vi "RemoteVI Server Share.vi"(0 "row":T1, 1 "port":u16=8100, 2 "whole network?":bool, 3 "view only?":bool, 8 "token":string) -> (4 "URL":string, 5 "message":string, 15 "error out":errorcluster)   [LabVIEW 2020, in "RemoteVI.lvlib"]
doc: "RemoteVI Server's Share button: shares the window of row. A panel of a RUNNING VI of this application instance (RemoteVI VI Of Window.vi) is shared as a VI target (RemoteVI Start.vi: tip strips and splitter dragging work); every other window - of another LabVIEW, a built application or any program, or the panel of a VI that is not running - as a window target (RemoteVI Start Window.vi). message is one line for the UI: the link, or why it failed (port in use, port shared already)."
uses:
  RemoteVI.lvlib
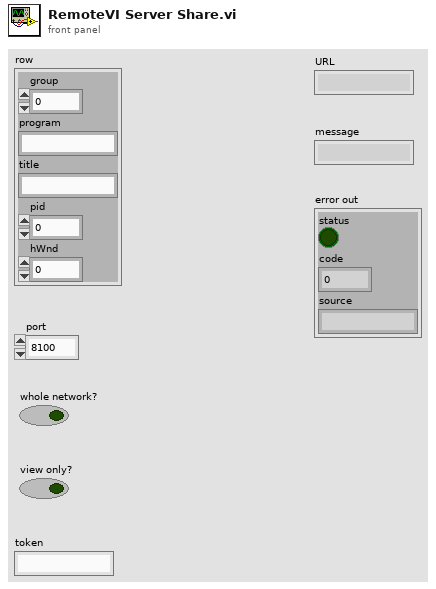
[diagram p1: front panel]
types:
  T1 = cluster{"group":i32, "program":string, "title":string, "pid":u32, "hWnd":u64}
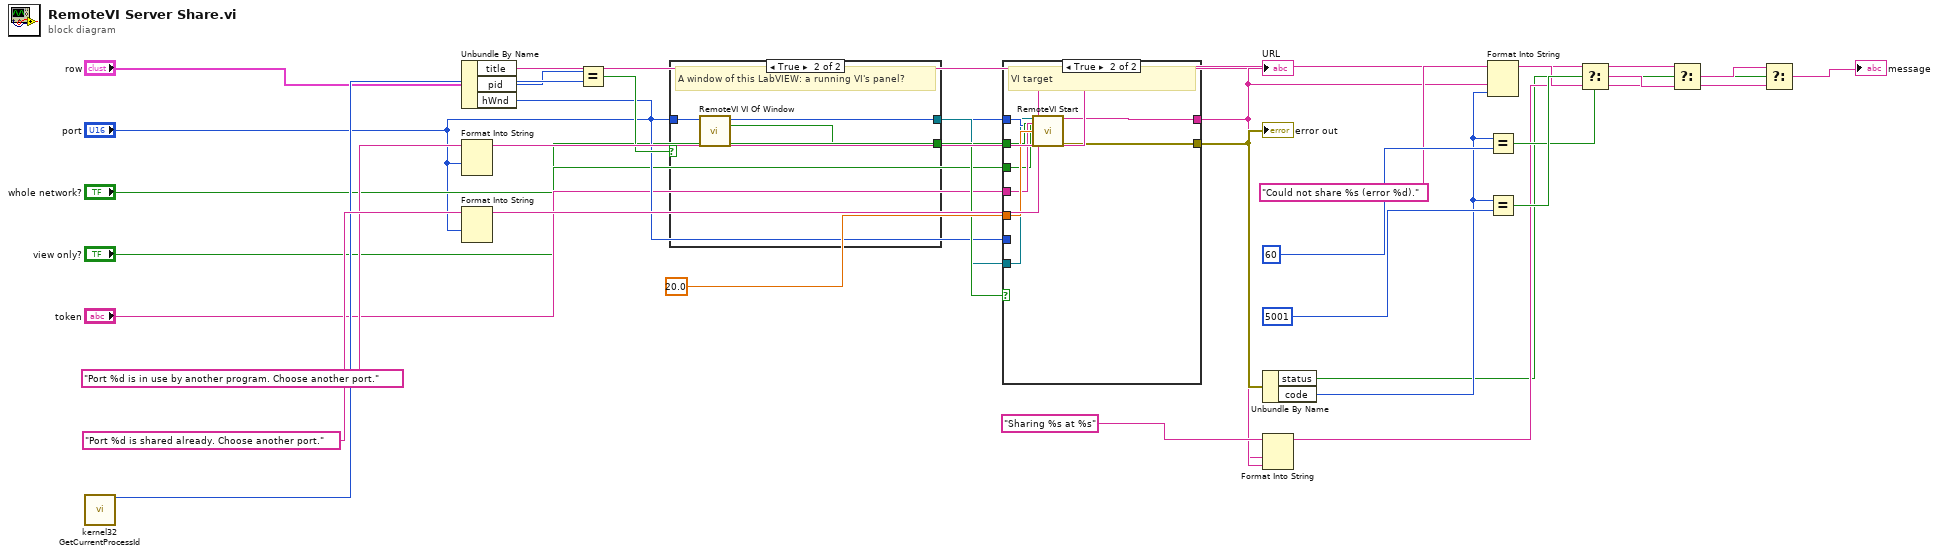
[diagram p0: block diagram]
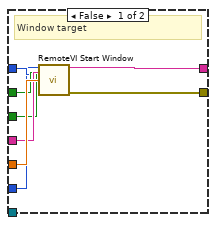
[diagram p2: hidden frame]
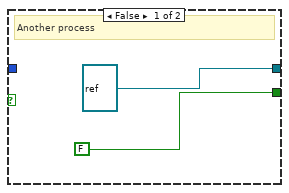
[diagram p3: hidden frame]
diagram:
  n1 = call "kernel32 GetCurrentProcessId.vi"() -> ("process ID"=w9:u32)  [unwired: 14 in, 1 out]
  n2 = Unbundle By Name("row") -> ("title"=w6:string, "pid"=w7:u32, "hWnd"=w8:u64)
  n3 = Format Into String(format string="Port %d is in use by another program. Choose another port.", "port") -> (resulting string=w21:string)  [unwired: 2 in, 1 out]
  n4 = Format Into String(format string="Port %d is shared already. Choose another port.", "port") -> (resulting string=w23:string)  [unwired: 2 in, 1 out]
  n5 = Equal?(x=w7, y=w9) -> (x = y?=w10:bool)
  n6 = case shown="True" w10 {
    tunnel: w8 -> [_ w35]
    tunnel: [refnum<vi> refnum w36] -> w11
    tunnel: [FALSE w37] -> w12
    frame False {
      # "Another process"
    }
    frame True {
      # "A window of this LabVIEW: a running VI's panel?"
      n7 = call "RemoteVI VI Of Window.vi"("window"=w35) -> ("VI"=w36:refnum<vi>, "found?"=w37:bool)  [unwired: 13 in]
    }
  }
  n8 = case shown="True" w12 {
    tunnel: "port" -> [w39 w47]
    tunnel: "whole network?" -> [w40 w48]
    tunnel: "view only?" -> [w41 w49]
    tunnel: "token" -> [w42 w50]
    tunnel: 20.0 -> [w43 w51]
    tunnel: w8 -> [w38 _]
    tunnel: w11 -> [_ w46]
    tunnel: [w44 w52] -> w14
    tunnel: [w45 w53] -> w15
    frame False {
      # "Window target"
      n9 = call "RemoteVI Start Window.vi"("window"=w38, "whole network?"=w40, "token"=w42, "view only?"=w41, "port"=w39, "fps"=w43) -> ("URL"=w44:string, "error out"=w45:errorcluster)  [unwired: 8 in]
    }
    frame True {
      # "VI target"
      n10 = call "RemoteVI Start.vi"("VI"=w46, "whole network?"=w48, "token"=w50, "view only?"=w49, "port"=w47, "fps"=w51) -> ("URL"=w52:string, "error out"=w53:errorcluster)  [unwired: 8 in]
    }
  }
  "URL" <- w14
  "error out" <- w15
  n11 = Unbundle By Name(w15) -> ("status"=w16:bool, "code"=w17:i32)
  n12 = Format Into String(format string="Sharing %s at %s", w6, w14) -> (resulting string=w19:string)  [unwired: 2 in, 1 out]
  n13 = Format Into String(format string="Could not share %s (error %d).", w6, w17) -> (resulting string=w25:string)  [unwired: 2 in, 1 out]
  n14 = Equal?(x=w17, y=60) -> (x = y?=w28:bool)
  n15 = Equal?(x=w17, y=5001) -> (x = y?=w29:bool)
  n16 = Select(t=w23, s=w29, f=w25) -> (s? t:f=w30:string)
  n17 = Select(t=w21, s=w28, f=w30) -> (s? t:f=w31:string)
  n18 = Select(t=w31, s=w16, f=w19) -> (s? t:f=→"message":string)
